vi "Create One Column Table HTML From Channel List.vi"(8 "Node#":i32, 9 "Color":string="invis", 10 "Title":string, 11 "display strings and indices":T1(array[cluster])) -> (2 "Table HTML":string, 3 "Channel and Node Pairs":T2[](array[typedef]))   [LabVIEW 2014, in "GraphViz Mapping Visualizer.lvlib"]
uses:
  GraphViz Mapping Visualizer.lvlib
  Channel to Port Pair.ctl
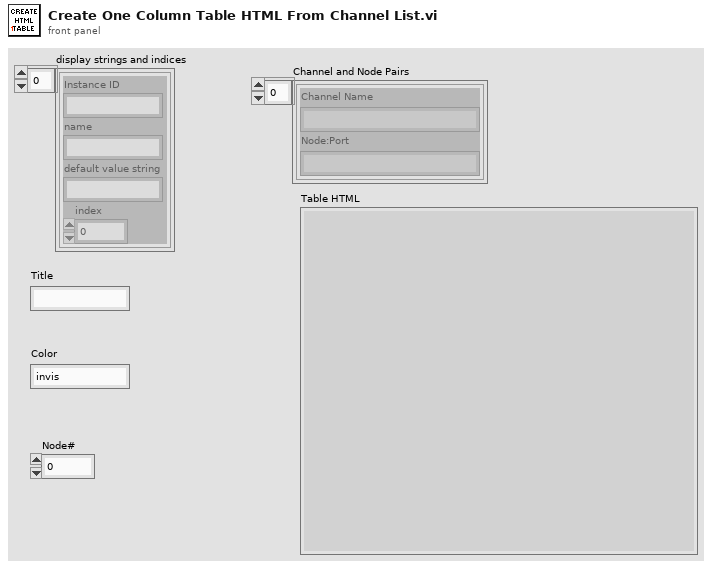
[diagram p1: front panel]
types:
  T1 = cluster{"Instance ID":string, "name":string, "default value string":string, "index":i32}[]
  T2 = typedef "GraphViz Mapping Visualizer.lvlib/Channel to Port Pair.ctl" = cluster{"Channel Name":string, "Node:Port":string}
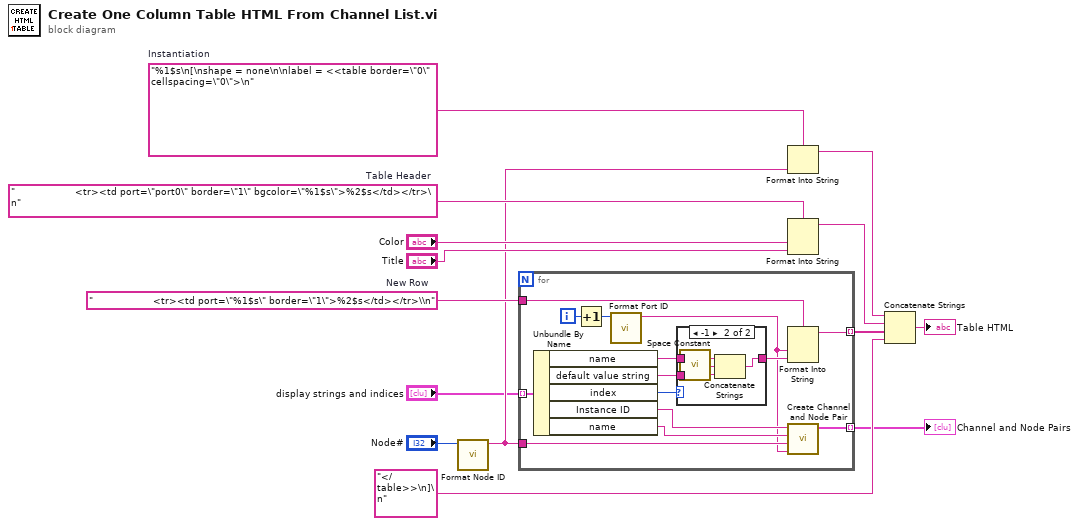
[diagram p0: block diagram]
diagram:
  w7 = "%1$s\n[\nshape = none\n\nlabel = <<table border=\"0\" cellspacing=\"0\">\n"  # Instantiation
  w12 = "                    <tr><td port=\"port0\" border=\"1\" bgcolor=\"%1$s\">%2$s</td></tr>\n"  # Table Header
  w14 = "                    <tr><td port=\"%1$s\" border=\"1\">%2$s</td></tr>\\n"  # New Row
  n1 = call "Format Node ID.vi"("node"="Node#") -> ("formatted node ID"=w2:string)  [unwired: 10 in]
  n2 = for {
    tunnel: [w27] -> w8 mode=indexing
    tunnel: w14 -> [w26]
    tunnel: w2 -> [w25]
    tunnel: [w24] -> w3 mode=indexing
    tunnel: "display strings and indices" -> [w23] mode=indexing
    i -> [w28]
    n3 = Unbundle By Name(w23) -> ("name"=w20:string, "default value string"=w19:string, "index"=w18:i32, "Instance ID"=w22:string, "name"=w21:string)
    n4 = Increment(x=w28) -> (x+1=w16:i32)
    n5 = call "Format Port ID.vi"("port"=w16) -> ("formatted port ID"=w15:string)  [unwired: 10 in]
    n6 = case shown="-1" w18 {
      tunnel: w20 -> [w29 w32]
      tunnel: w19 -> [_ w31]
      tunnel: [w29 w30] -> w17
      frame Default {
      }
      frame -1 {
        n7 = call <vilib>:"Space Constant.vi"() -> ("String"=w33:string)
        n8 = Concatenate Strings(w32, w33, w31) -> (w30:string)
      }
    }
    n9 = Format Into String(format string=w26, w15, w17) -> (resulting string=w27:string)  [unwired: 2 in, 1 out]
    n10 = call "Create Channel and Node Pair.vi"("Port ID"=w15, "Node ID"=w25, "name"=w21, "Instance ID"=w22) -> ("Channel to Port Pair"=w24:T2)  [unwired: 7 in]
  }
  "Channel and Node Pairs" <- w3
  n11 = Format Into String(format string=w7, w2) -> (resulting string=w6:string)  [unwired: 2 in, 1 out]
  n12 = Format Into String(format string=w12, "Color", "Title") -> (resulting string=w9:string)  [unwired: 2 in, 1 out]
  n13 = Concatenate Strings(w6, w9, w8, "</table>>\n]\n") -> (→"Table HTML":string)
